vi "test Find Disabled Custom Devices.vi"(8 "error in":errorcluster, 11 "TestCase in":refnum<class "Scripting.lvclass">) -> (0 "error out":errorcluster, 3 "TestCase out":refnum<class "Scripting.lvclass">)   [LabVIEW 2020, in "Scripting.lvclass"]
uses:
  Scripting.lvclass
  Scripting.lvclass/Scripting.ctl
  Scripting/Ballard/Ballard ARINC 429 Scripting.lvlib
  <vilib>/addons/_JKI Toolkits/VI Tester/TestCase.llb/TestCase.lvclass
  C:/Program Files (x86)/National Instruments/LabVIEW 2020/vi.lib/addons/_JKI Toolkits/VI Tester/TestCase.llb/TestCase.lvclass
  C:/dev/git/niveristand-ballard-arinc429-custom-device/Source/Custom Device Support/Tests/Unit/Scripting/Scripting.lvclass
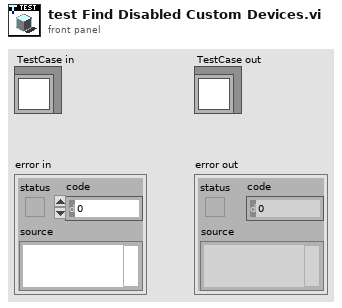
[diagram p1: front panel]
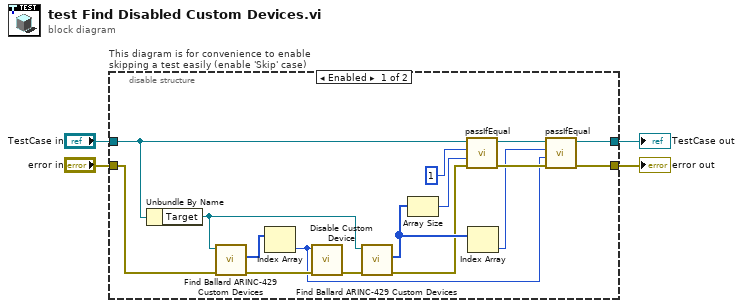
[diagram p0: block diagram]
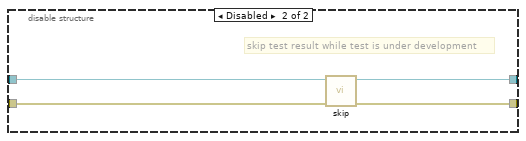
[diagram p2: hidden frame]
diagram:
  n1 = disable-structure "This diagram is for convenience to enable skipping a test easily (enable 'Skip' case)" shown="Enabled" {
    disable-tunnel: "TestCase in" -> [w16 w24]
    disable-tunnel: [w9 w22] -> w4
    disable-tunnel: [w5 w23] -> w2
    disable-tunnel: "error in" -> [w20 w21]
    frame Enabled {
      n2 = Unbundle By Name(w16) -> ("Target"=w14:refnum<k24>)
      n3 = call "Find Ballard ARINC-429 Custom Devices.vi"("error in"=w20, "target in"=w14) -> ("error out"=w17:errorcluster, "Ballard ARINC 429 custom devices"=w18:u64[])  [unwired: 7 in, 1 out]
      n4 = Index Array(array=w18) -> (element=w7:u64)  [unwired: 1 in]
      n5 = call "Disable Custom Device.vi"("error in (no error)"=w17, "Ballard ARINC 429 ref"=w7) -> ("error out"=w15:errorcluster)  [unwired: 8 in, 1 out]
      n6 = call "Find Ballard ARINC-429 Custom Devices.vi"("error in"=w15, "target in"=w14) -> ("error out"=w6:errorcluster, "Ballard ARINC 429 custom devices"=w11:u64[])  [unwired: 7 in, 1 out]
      n7 = Array Size(array=w11) -> (size(s)=w12:i32)
      n8 = call-dynamic "passIfEqual.vi"("error in (no error)"=w6, "y"=w12, "x"=1, "TestCase in"=w16) -> ("error out"=w19:errorcluster, "TestCase out"=w10:refnum<class "Scripting.lvclass">)  [unwired: 6 in]
      n9 = Index Array(array=w11) -> (element=w8:u64)  [unwired: 1 in]
      n10 = call-dynamic "passIfEqual.vi"("error in (no error)"=w19, "y"=w7, "x"=w8, "TestCase in"=w10) -> ("error out"=w5:errorcluster, "TestCase out"=w9:refnum<class "Scripting.lvclass">)  [unwired: 6 in]
    }
    frame Disabled {
      # "skip test result while test is under development"
      n11 = call <vilib>:"skip.vi"("error in (no error)"=w21, "TestCase in"=w24) -> ("error out"=w23:errorcluster, "TestCase out"=w22:refnum<class "Scripting.lvclass">)  [unwired: 8 in]
    }
  }
  "error out" <- w2
  "TestCase out" <- w4
